vi "Initialize.vi"(5 "Operation Interface in":refnum<class "Program Interface.lvclass">) -> (19 "Operation Interface out":refnum<class "Program Interface.lvclass">)   [LabVIEW 2019, in "Program Interface.lvclass"]
uses:
  Program Interface.lvclass
  Program Interface.lvclass/Program Interface.ctl
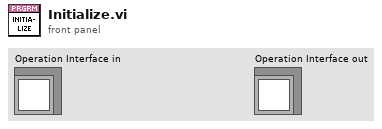
[diagram p1: front panel]
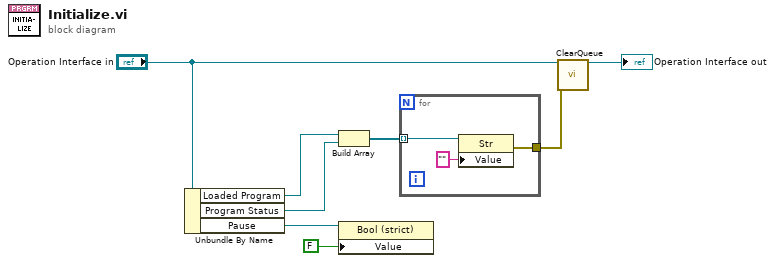
[diagram p0: block diagram]
diagram:
  n1 = Unbundle By Name("Operation Interface in") -> ("Loaded Program"=w8:refnum<vi>, "Program Status"=w7:refnum<vi>, "Pause"=w2:refnum<vi>)
  n2 = Build Array(w8, w7) -> (w6:refnum<vi>[])
  n3 = property class="Bool (strict)"(reference=w2, "Value"=FALSE) -> ()  [unwired: 1 in, 2 out]
  n4 = for {
    tunnel: w6 -> [w11] mode=indexing
    tunnel: [w9] -> w3
    n5 = property class="Str"(reference=w11, "Value"="") -> (error out=w9:errorcluster)  [unwired: 1 in, 1 out]
  }
  n6 = call "ClearQueue.vi"("Program Interface in"="Operation Interface in", "error in (no error)"=w3) -> ("Program Interface out"=→"Operation Interface out":refnum<class "Program Interface.lvclass">)  [unwired: 16 in, 1 out]
